vi "Delete.vi"(8 "error in (no error)":errorcluster, 11 "ARN in":refnum<class "ARN.lvclass">) -> (0 "error out":errorcluster)   [LabVIEW 2015, in "NI_AWS_Core.lvlib" / "ARN.lvclass"]
uses:
  ARN.lvclass
  HTTP Request/Name Value Pair.ctl
  HTTP Request/HTTP Request.lvclass
  HTTP Request/Request Options.ctl
  HTTP Request/Region handling.ctl
  HTTP Request/URL formatting.ctl
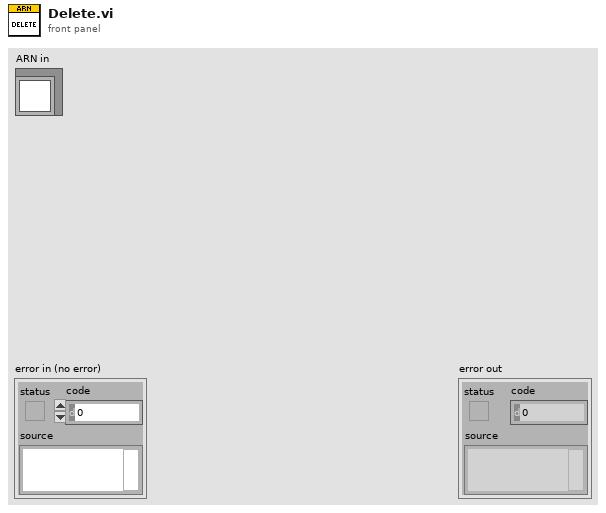
[diagram p1: front panel]
types:
  T1 = typedef "NI_AWS_Core.lvlib/HTTP Request.lvclass/Request Options.ctl" = cluster{"request headers":T2[], "request parameters":T2[], "request body":string, "region handling":T3, "URL formatting":T4}
  T2 = typedef "NI_AWS_Core.lvlib/HTTP Request.lvclass/Name Value Pair.ctl" = cluster{"name":string, "value":string}
  T3 = typedef "NI_AWS_Core.lvlib/HTTP Request.lvclass/Region handling.ctl" = enum16{"use region everywhere", "use region (authentication only)", "use region (URL only)", "ignore region everwhere"}
  T4 = typedef "NI_AWS_Core.lvlib/HTTP Request.lvclass/URL formatting.ctl" = enum16{"region-", "region."}
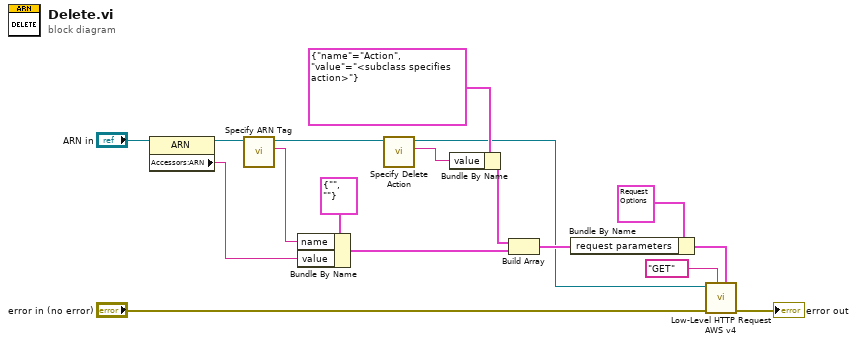
[diagram p0: block diagram]
diagram:
  n1 = property class="ARN"(reference="ARN in") -> (reference out=w10:refnum<class "ARN.lvclass">, "Accessors:ARN"=w14:string)  [unwired: 1 in, 1 out]
  n2 = call-dynamic "Specify ARN Tag.vi"("ARN in"=w10) -> ("ARN Tag"=w9:string, "ARN out"=w8:refnum<class "ARN.lvclass">)  [unwired: 9 in]
  n3 = Bundle By Name(cluster=T2 {"name"="", "value"=""} ("element"), "name"=w9, "value"=w14) -> (w16:T2)
  n4 = call-dynamic "Specify Delete Action.vi"("ARN in"=w8) -> ("Delete action"=w7:string, "ARN out"=w1:refnum<class "ARN.lvclass">)  [unwired: 9 in]
  n5 = Bundle By Name(cluster=T2 {"name"="Action", "value"="<subclass specifies action>"} ("Name Value Pair"), "value"=w7) -> (w5:T2)
  n6 = Build Array(w5, w16) -> (w15:T2[])
  n7 = Bundle By Name(cluster=T1 {"request headers"=[], "request parameters"=[], "request body"="", "region handling"=enum."use region everywhere", "URL formatting"=enum."region."} ("Request Options"), "request parameters"=w15) -> (w3:T1)
  n8 = call "Low-Level HTTP Request AWS v4.vi"("Request Options"=w3, "HTTP-Verb"="GET", "error in (no error)"="error in (no error)", "AWS Core in"=w1) -> ("error out"=→"error out":errorcluster)  [unwired: 4 in, 3 out]
